vi "AttachThreadInput Wrapper Template.vi"(0 "idAttach":u32, 5 "idAttachTo":u32, 7 "fAttach":i32=1, 11 "error in":errorcluster) -> (4 "return value":i32, 15 "error out":errorcluster)   [LabVIEW 2020]
doc: "Attaches (fAttach non-zero) or detaches (0) the input processing of thread idAttach to that of thread idAttachTo through user32.dll AttachThreadInput (stdcall, called in LabVIEW's UI thread). While attached, both threads share one key state, so user32 SetKeyboardState.vi called in the UI thread writes the key state the other thread reads. return value is the Win32 BOOL: non-zero on success. When error in carries an error the DLL is not called. Generated by tools\\Build Win32 Wrappers.vi - do not edit by hand, rebuild it."
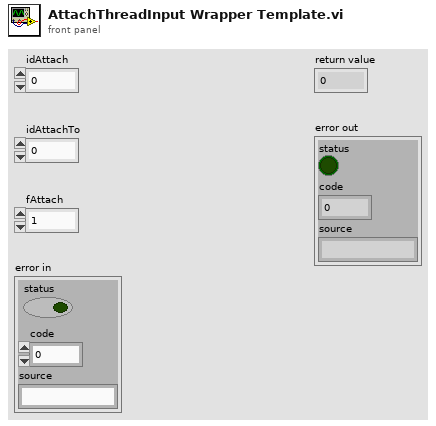
[diagram p1: front panel]
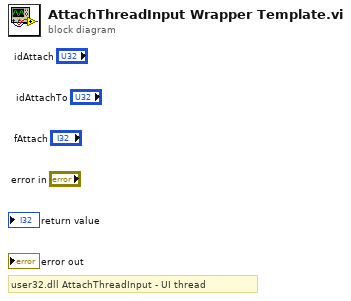
[diagram p0: block diagram]
diagram:
  # "user32.dll AttachThreadInput - UI thread"
